vi "VIH HelpGen - Close VI Reference.vi"(8 "error in":errorcluster, 11 "VI Reference":refnum<vi>) -> (0 "error out":errorcluster)   [LabVIEW 2014]
doc: "::: VI Helpeks :::\nCopyright (c) 2000-2026 Konstantin Shifershteyn. All rights reserved."
panel:
  # "VI Helpeks\nCopyright (c) 2012-2026 Konstantin Shifershteyn"
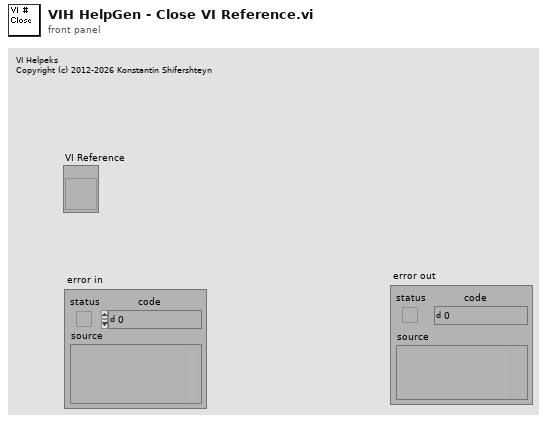
[diagram p1: front panel]
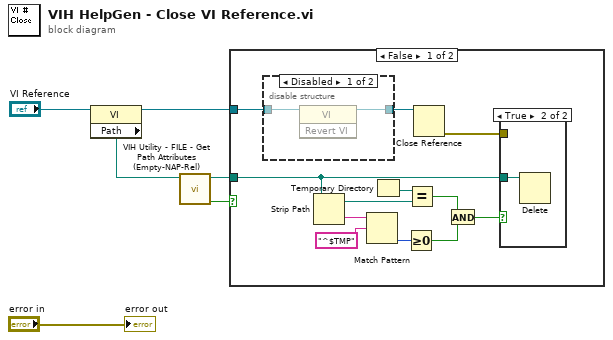
[diagram p0: block diagram]
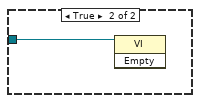
[diagram p4: hidden frame]
diagram:
  n1 = property class="VI"(reference="VI Reference") -> (reference out=w1:refnum<vi>, "Path"=w4:path)  [unwired: 1 in, 1 out]
  n2 = call "VIH Utility - FILE - Get Path Attributes (Empty-NAP-Rel).vi"("Path"=w4) -> ("Not A Path or Empty path"=w2:bool, "dup Path"=w3:path)  [unwired: 6 in, 3 out]
  n3 = case shown="False" w2 {
    tunnel: w1 -> [w8 w23]
    tunnel: w3 -> [w9 _]
    frame False {
      n4 = disable-structure shown="Disabled" {
        disable-tunnel: w8 -> [w20 w21]
        disable-tunnel: [w19 w21] -> w7
        frame Disabled {
          n5 = invoke class="VI" method="Revert VI"(reference=w20) -> (reference out=w19:refnum<vi>)  [unwired: 2 in, 2 out]
        }
        frame Enabled {
        }
      }
      n6 = Strip Path(path=w9) -> (stripped path=w14:path, name=w18:string)
      n7 = Match Pattern(string=w18, regular expression="^$TMP") -> (offset past match=w16:i32)  [unwired: 1 in, 3 out]
      n8 = Temporary Directory() -> (w13:path)
      n9 = Greater Or Equal To 0?(x=w16) -> (x >= 0?=w11:bool)
      n10 = Equal?(x=w13, y=w14) -> (x = y?=w12:bool)
      n11 = Close Reference(reference=w7) -> (error out=w15:errorcluster)  [unwired: 1 in]
      n12 = And(x=w12, y=w11) -> (x .and. y?=w10:bool)
      n13 = case shown="True" w10 {
        tunnel: w9 -> [_ w22]
        tunnel: w15 -> [_ _]
        frame False {
        }
        frame True {
          n14 = Delete(path (use dialog)=w22) -> ()  [unwired: 4 in, 3 out]
        }
      }
    }
    frame True {
      n15 = invoke class="VI" method="Empty"(reference=w23) -> ()  [unwired: 2 in, 3 out]
    }
  }
  "error out" <- "error in"
